vi "Compare New Values.vi"(8 "error in (no error)":errorcluster, 10 "New Values":string[](array[string]), 11 "Selector in":refnum<class "Selector.lvclass">) -> (0 "error out":errorcluster, 2 "Unchanged ?":bool, 3 "Selector out":refnum<class "Selector.lvclass">)   [LabVIEW 2019, in "Selector.lvclass"]
uses:
  Selector.lvclass
  Selector.lvclass/Selector.ctl
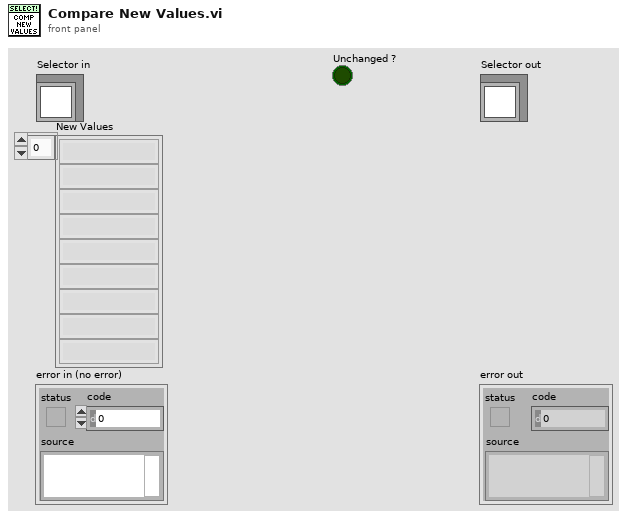
[diagram p1: front panel]
types:
  T1 = typedef "Selector.lvclass/Item.ctl" = cluster{"Name":string, "Group":string, "Enabled":bool}
  T2 = cluster{"Name":string, "Group":string, "Enabled":bool}
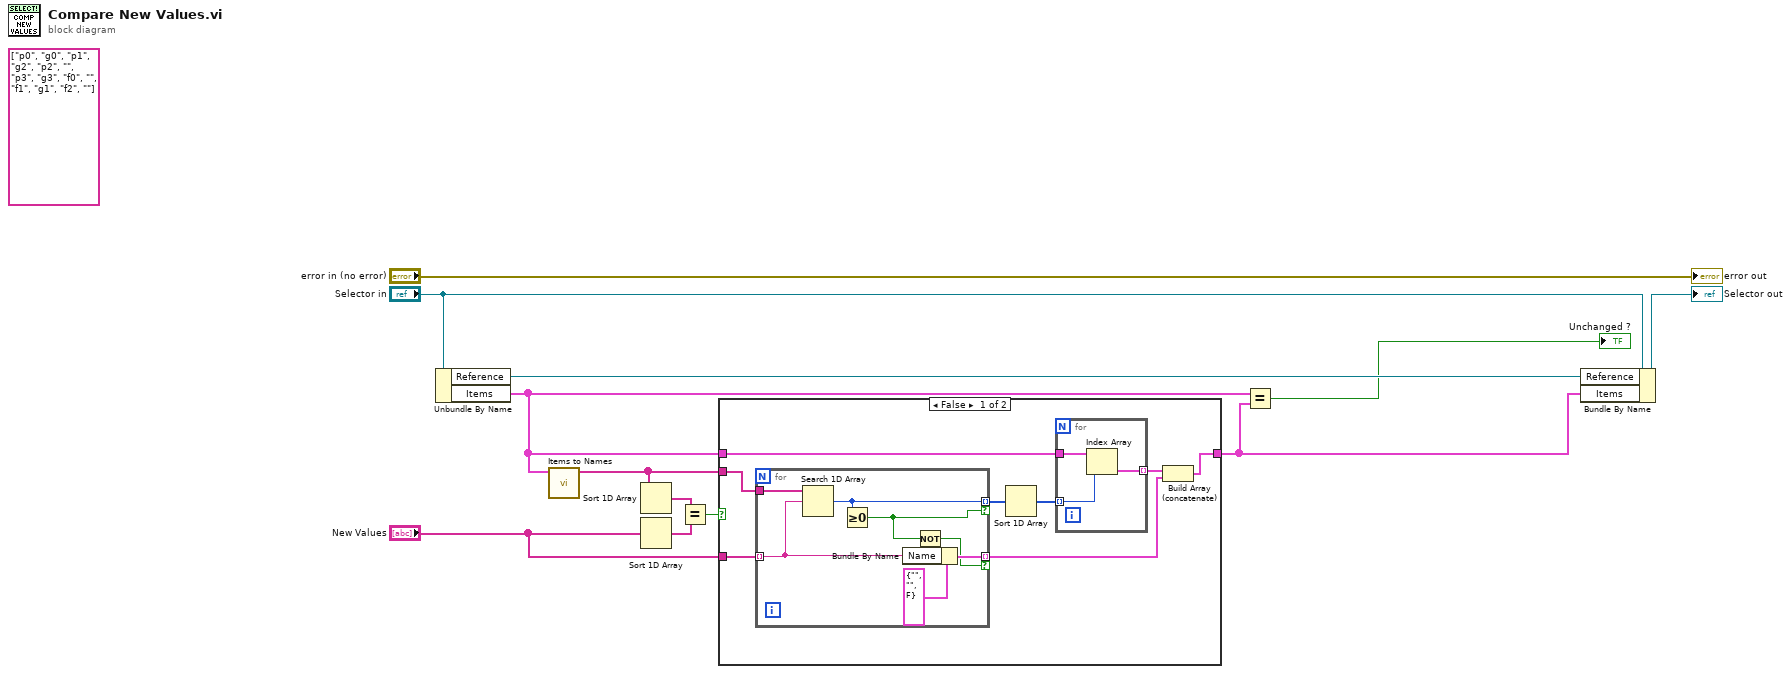
[diagram p0: block diagram]
diagram:
  (unwired) string[][] [["p0", "g0"], ["p1", "g2"], ["p2", ""], ["p3", "g3"], ["f0", ""], ["f1", "g1"], ["f2", ""]] ("Item Names")
  n1 = Unbundle By Name("Selector in") -> ("Reference"=w3:refnum<vi>, "Items"=w7:T1[])
  n2 = call "Items to Names.vi"("Items"=w7) -> ("Names"=w9:string[])  [unwired: 6 in]
  n3 = Sort 1D Array(array=w9) -> (sorted array=w12:string[])
  n4 = Sort 1D Array(array="New Values") -> (sorted array=w11:string[])
  n5 = Equal?(x=w12, y=w11) -> (x = y?=w10:bool)
  n6 = case shown="False" w10 {
    tunnel: w7 -> [w17 w31]
    tunnel: w9 -> [w20 _]
    tunnel: "New Values" -> [w19 _]
    tunnel: [w13 w31] -> w2
    frame False {
      n7 = for {
        tunnel: w20 -> [w30]
        tunnel: w19 -> [w26] mode=indexing
        tunnel: [w28] -> w18 mode=indexing if=w24
        tunnel: [w27] -> w14 mode=indexing if=w25
        n8 = Search 1D Array(1D array=w30, element=w26) -> (index of element=w28:i32)  [unwired: 1 in]
        n9 = Greater Or Equal To 0?(x=w28) -> (x >= 0?=w24:bool)
        n10 = Bundle By Name(cluster=T2 {"Name"="", "Group"="", "Enabled"=FALSE} ("Item"), "Name"=w26) -> (w27:T2)
        n11 = Not(x=w24) -> (.not. x?=w25:bool)
      }
      n12 = Sort 1D Array(array=w18) -> (sorted array=w16:i32[])
      n13 = for {
        tunnel: w17 -> [w23]
        tunnel: w16 -> [w22] mode=indexing
        tunnel: [w21] -> w15 mode=indexing
        n14 = Index Array(array=w23, index=w22) -> (element=w21:T1)
      }
      n15 = Build Array (concatenate)(w15, w14) -> (w13:T1[])
    }
    frame True {
    }
  }
  n16 = Equal?(x=w7, y=w2) -> (x = y?=→"Unchanged ?":bool)
  n17 = Bundle By Name(cluster="Selector in", "Reference"=w3, "Items"=w2) -> (→"Selector out":refnum<class "Selector.lvclass">)
  "error out" <- "error in (no error)"
